vi "Diff_Drive_System_Act_AutoTune.vi"(6 "FPGA_Time_Seconds":dbl, 7 "Enabled":bool=TRUE, 9 "Right Speed":dbl, 10 "Left Speed":dbl, 11 "Diff_Drive_Device_Refs":T1 {"GyroDevRef"."Sample Rate" min=0.25 max=100.0 step=0.25}) -> ()   [LabVIEW 2019]
uses:
  <vilib>/Rock Robotics/WPI/ThirdParty/JAS_Junk/TrajLib/Trajectory_Library.lvlib
  Diff_Drive_System_Globals.vi
  <vilib>/Rock Robotics/SystemInterfaces/DIO/FPGA_DIOPWMChannel.ctl
  <vilib>/Rock Robotics/WPI/PWM/WPI_PWMDeadband.ctl
  <vilib>/Rock Robotics/WPI/MotorControl/WPI_MotorControlType.ctl
  <vilib>/Rock Robotics/SystemInterfaces/DIO/FPGA_DIOChannel.ctl
  <vilib>/Rock Robotics/WPI/MotorControl/WPI_MotorControlDeviceRef.ctl
  <vilib>/Rock Robotics/WPI/RobotDrive/WPI_RobotDriveDevRef.ctl
  <vilib>/Rock Robotics/SystemInterfaces/Encoder/FPGA_EncoderIdx.ctl
  <vilib>/Rock Robotics/WPI/Encoder/WPI_EncoderType.ctl
  <vilib>/Rock Robotics/SystemInterfaces/Counter/FPGA_CounterCtrSystemIndex.ctl
  <vilib>/Rock Robotics/WPI/Encoder/WPI_EncoderDevRef.ctl
  <vilib>/Rock Robotics/SystemInterfaces/spilib/spi_bus.ctl
  <vilib>/Rock Robotics/SystemInterfaces/AI/FPGA_AIChannel.ctl
  <vilib>/Rock Robotics/WPI/Gyro/WPI_GyroDevRef.ctl
  Diff_Drive_System_Device_Refs.ctl
panel:
  # "Analog"
  # "XRS"
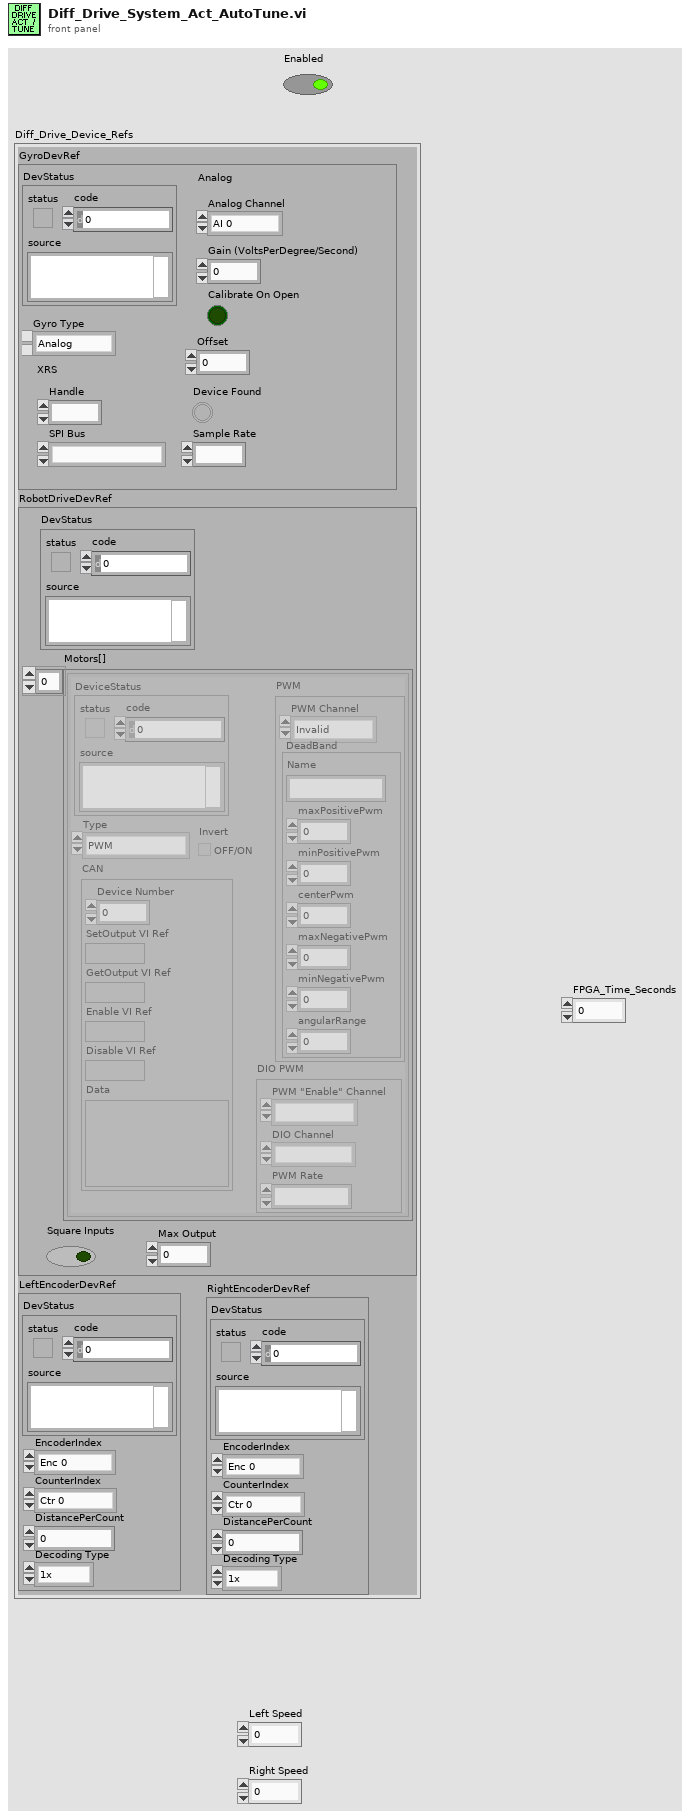
[diagram p1: front panel]
types:
  T1 = typedef "Diff_Drive_System_Device_Refs.ctl" = cluster{"GyroDevRef":T2, "RobotDriveDevRef":T5, "LeftEncoderDevRef":T11, "RightEncoderDevRef":T11}
  T2 = typedef "WPI_GyroDevRef.ctl" = cluster{"DevStatus":errorcluster, "Analog Channel":T3, "Gain (VoltsPerDegree/Second)":dbl, "Gyro Type":enum16{"Analog", "XRS450"}, "Handle":i32, "SPI Bus":T4, "Device Found":bool, "Sample Rate":dbl, "Calibrate On Open":bool, "Offset":dbl}
  T3 = typedef "FPGA_AIChannel.ctl" = enum8{"AI 0", "AI 1", "AI 2", "AI 3", "AI MXP 0", "AI MXP 1", "AI MXP 2", "AI MXP 3", "Invalid"}
  T4 = typedef "spi_bus.ctl" = enum16{"SPI On-Board, CS0", "SPI On-Board, CS1", "SPI On-Board, CS2", "SPI On-Board, CS3", "SPI MXP", "Invalid"}
  T5 = typedef "WPI_RobotDriveDevRef.ctl" = cluster{"DevStatus":errorcluster, "Motors[]":T6[], "Square Inputs":bool, "Max Output":dbl}
  T6 = typedef "WPI_MotorControlDeviceRef.ctl" = cluster{"DeviceStatus":errorcluster, "Type":T7, "PWM":cluster{"PWM Channel":T8, "DeadBand":T9}, "CAN":cluster{"Device Number":u8, "SetOutput VI Ref":variant, "GetOutput VI Ref":variant, "Enable VI Ref":variant, "Disable VI Ref":variant, "Data":variant}, "Invert":bool, "DIO PWM":cluster{"PWM \"Enable\" Channel":T8, "DIOChannel":T10, "PWM Rate":dbl}}
  T7 = typedef "WPI_MotorControlType.ctl" = enum16{"PWM", "CAN", "DIO PWM"}
  T8 = typedef "FPGA_DIOPWMChannel.ctl" = enum8{"PWM 0", "PWM 1", "PWM 2", "PWM 3", "PWM 4", "PWM 5", "PWM 6", "PWM 7", "PWM 8", "PWM 9", "PWM MXP 0", "PWM MXP 1", "PWM MXP 2", "PWM MXP 3", "PWM MXP 4", "PWM MXP 5", "PWM MXP 6", "PWM MXP 7", "PWM MXP 8", "PWM MXP 9", "Invalid"}
  T9 = typedef "WPI_PWMDeadband.ctl" = cluster{"Name":string, "maxPositivePwm":i32, "minPositivePwm":i32, "centerPwm":i32, "maxNegativePwm":i32, "minNegativePwm":i32, "angularRange":u16}
  T10 = typedef "FPGA_DIOChannel.ctl" = enum8{"DIO 0", "DIO 1", "DIO 2", "DIO 3", "DIO 4", "DIO 5", "DIO 6", "DIO 7", "DIO 8", "DIO 9", "DIO MXP 0", "DIO MXP 1", "DIO MXP 2", "DIO MXP 3", "DIO MXP 4", "DIO MXP 5", "DIO MXP 6", "DIO MXP 7", "DIO MXP 8", "DIO MXP 9", "DIO MXP 10", "DIO MXP 11", "DIO MXP 12", "DIO MXP 13", "DIO MXP 14", "DIO MXP 15", "SPI Port CS1", "SPI Port CS2", "SPI Port CS3", "SPI Port MISO", "SPI Port MOSI", "Invalid"}
  T11 = typedef "WPI_EncoderDevRef.ctl" = cluster{"DevStatus":errorcluster, "EncoderIndex":T12, "CounterIndex":T13, "DistancePerCount":dbl, "Decoding Type":T14}
  T12 = typedef "FPGA_EncoderIdx.ctl" = enum8{"Enc 0", "Enc 1", "Enc 2", "Enc 3", "Enc 4", "Enc 5", "Enc 6", "Enc 7", "Invalid"}
  T13 = typedef "FPGA_CounterCtrSystemIndex.ctl" = enum8{"Ctr 0", "Ctr 1", "Ctr 2", "Ctr 3", "Ctr 4", "Ctr 5", "Ctr 6", "Ctr 7", "Invalid"}
  T14 = typedef "WPI_EncoderType.ctl" = enum16{"1x", "2x", "4x"}
  T15 = enum16{"Ziegler Nicols - Fast", "Ziegler Nicols - Normal", "Ziegler Nicols - Slow", "CHR regulator - 0% overshoot", "CHR regulator - 20% overshoot", "CHR servo - 0 % overshoot", "CHR servo - 20% overshoot"}
  T16 = typedef "Trajectory_Library.lvlib/SIMPLE_MOTOR_FF.ctl" = cluster{"Ks":dbl, "Kv":dbl, "Ka":dbl, "KnInv":dbl}
  T17 = typedef "Trajectory_Library.lvlib/PID_ADV_LIMITS.ctl" = cluster{"MaxInput":dbl, "MinInput":dbl, "Continuous":bool, "MaxOutput":dbl, "MinOutput":dbl}
  T18 = typedef "Trajectory_Library.lvlib/PID_ADV_TUNING.ctl" = cluster{"Kf":dbl, "Kp":dbl, "Ki":dbl, "Kd":dbl, "MaximumIntegral":dbl, "MinimumIntegral":dbl, "Filter Derivative":bool}
  T19 = cluster{"Controller Constant Type":enum16{"Ziegler Nicols - Fast", "Ziegler Nicols - Normal", "Ziegler Nicols - Slow", "CHR regulator - 0% overshoot", "CHR regulator - 20% overshoot", "CHR servo - 0 % overshoot", "CHR servo - 20% overshoot"}, "Type of Controller":enum16{"P", "PI", "PID"}, "CO Offset":dbl, "Kn":dbl, "Tuning Tolerance":dbl, "Plant Tolerance":dbl, "Newest Avg Time ":i32, "Long Ave Time":i32}
  T20 = cluster{"proportional gain (Kp)":dbl, "integral time (Ki / Sec)":dbl, "derivative time (Kd /Sec)":dbl}
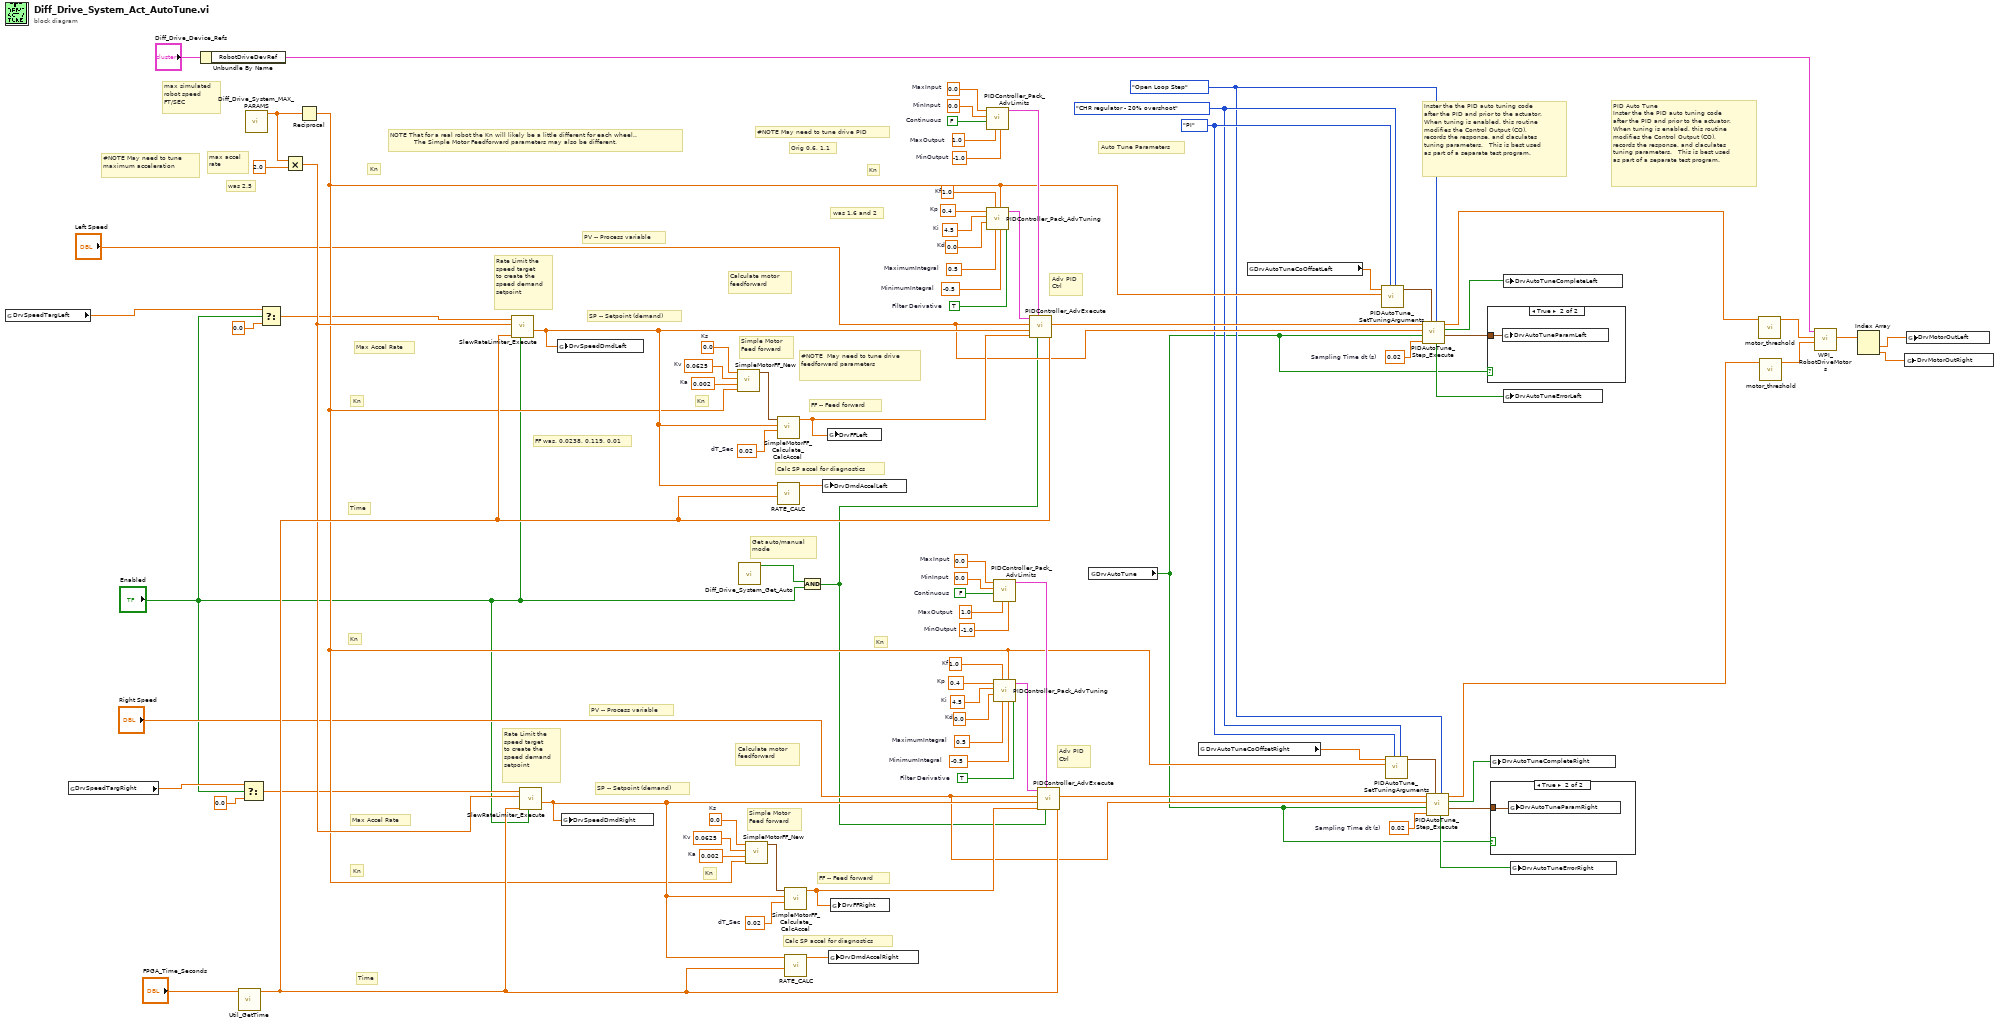
[diagram p0: block diagram]
diagram:
  w28 = 0.02  # Sampling Time dt (s)
  w13 = enum16{"Open Loop Step", "Closed Loop Step"}."Open Loop Step" ("Procedure Type")
  w14 = T15."CHR regulator - 20% overshoot" ("Controller Constant Type")
  w15 = enum16{"P", "PI", "PID"}."PI" ("Type of Controller")
  w33 = 0.02  # Sampling Time dt (s)
  w52 = 0.4  # Kp
  w51 = 4.5  # Ki
  w50 = 0.0  # Kd
  w49 = 1.0  # Kf
  w48 = 0.5  # MaximumIntegral
  w47 = -0.5  # MinimumIntegral
  w46 = TRUE  # Filter Derivative
  w44 = 0.0  # MinInput
  w43 = FALSE  # Continuous
  w42 = 1.0  # MaxOutput
  w45 = -1.0  # MinOutput
  w41 = 0.0  # MaxInput
  w57 = 0.02  # dT_Sec
  w55 = 0.0  # Ks
  w54 = 0.0625  # Kv
  w53 = 0.002  # Ka
  w75 = 0.4  # Kp
  w74 = 4.5  # Ki
  w73 = 0.0  # Kd
  w72 = 1.0  # Kf
  w71 = 0.5  # MaximumIntegral
  w70 = -0.5  # MinimumIntegral
  w69 = TRUE  # Filter Derivative
  w67 = 0.0  # MinInput
  w66 = FALSE  # Continuous
  w65 = 1.0  # MaxOutput
  w68 = -1.0  # MinOutput
  w64 = 0.0  # MaxInput
  w80 = 0.02  # dT_Sec
  w78 = 0.0  # Ks
  w77 = 0.0625  # Kv
  w76 = 0.002  # Ka
  # "PID Auto Tune\nInster the the PID auto tuning code\nafter the PID and prior to the actuator.\nWhen tuning is enabled, this routine\nmodifies the Control Output (CO), \nrecords the response, and claculates\ntuning parameters.   This is best used\nas part of a separate test program."
  # "was 1.6 and 2"
  # "Auto Tune Parameters"
  # "Inster the the PID auto tuning code\nafter the PID and prior to the actuator.\nWhen tuning is enabled, this routine\nmodifies the Control Output (CO), \nrecords the response, and claculates\ntuning parameters.   This is best used\nas part of a separate test program."
  # "Get auto/manual\nmode"
  # "FF was, 0.0238, 0.119, 0.01"
  # "Orig 0.6, 1.1"
  # "NOTE That for a real robot the Kn will likely be a little different for each wheel..\n            The Simple Motor Feedforward parameters may also be different."
  # "Max Accel Rate"
  # "Max Accel Rate"
  # "Time"
  # "Kn"
  # "Kn"
  # "Kn"
  # "Kn"
  # "Time"
  # "Kn"
  # "PV -- Process variable"
  # "Kn"
  # "Calc SP accel for diagnostics"
  # "FF -- Feed forward"
  # "SP -- Setpoint (demand)"
  # "Adv PID\nCtrl"
  # "Calculate motor\nfeedforward"
  # "Rate Limit the \nspeed target\nto create the\nspeed demand\nsetpoint"
  # "Simple Motor\nFeed forward"
  # "Kn"
  # "PV -- Process variable"
  # "Kn"
  # "Calc SP accel for diagnostics"
  # "FF -- Feed forward"
  # "SP -- Setpoint (demand)"
  # "Adv PID\nCtrl"
  # "Calculate motor\nfeedforward"
  # "was 2.5"
  # "Rate Limit the \nspeed target\nto create the\nspeed demand\nsetpoint"
  # "Simple Motor\nFeed forward"
  # "#NOTE May need to tune drive PID"
  # "#NOTE May need to tune maximum acceleration"
  # "#NOTE  May need to tune drive feedforward parameters"
  # "max simulated\nrobot speed\nFT/SEC"
  # "max accel\nrate"
  n1 = global read "Diff_Drive_System_Globals.vi" "DrvSpeedTargLeft"() -> (w4:dbl)
  n2 = global read "Diff_Drive_System_Globals.vi" "DrvSpeedTargRight"() -> (w6:dbl)
  n3 = Unbundle By Name("Diff_Drive_Device_Refs") -> ("RobotDriveDevRef"=w83:T5)
  n4 = call <vilib>:"Util_GetTime.vi"("Pass_Through_Time"="FPGA_Time_Seconds") -> ("FPGA_Time_Seconds"=w38:dbl)  [unwired: 8 in, 2 out]
  n5 = Select(t=w6, s="Enabled", f=0.0) -> (s? t:f=w7:dbl)
  n6 = call "Diff_Drive_System_MAX_PARAMS.vi"() -> ("Max Speed Ft/Sec"=w59:dbl)  [unwired: 9 in, 2 out]
  n7 = Select(t=w4, s="Enabled", f=0.0) -> (s? t:f=w3:dbl)
  n8 = Multiply(x=w59, y=2.0 ("x")) -> (x*y=w37:dbl)
  n9 = Reciprocal(x=w59) -> (1/x=w23:dbl)
  n10 = call <vilib>:"SlewRateLimiter_Execute.vi"("Enable"="Enabled", "Time"=w38, "PositiveRate"=w37, "Input"=w3) -> ("Output"=w61:dbl)  [unwired: 6 in, 1 out]
  n11 = call <vilib>:"SlewRateLimiter_Execute.vi"("Enable"="Enabled", "Time"=w38, "PositiveRate"=w37, "Input"=w7) -> ("Output"=w34:dbl)  [unwired: 6 in, 1 out]
  n12 = global write "Diff_Drive_System_Globals.vi" "DrvSpeedDmdLeft"(w61) -> ()
  n13 = global write "Diff_Drive_System_Globals.vi" "DrvSpeedDmdRight"(w34) -> ()
  n14 = call <vilib>:"SimpleMotorFF_New.vi"("Kn"=w23, "Ka"=w76, "Kv"=w77, "Ks"=w78) -> ("SIMPLE_MOTOR_FF"=w79:T16)  [unwired: 7 in]
  n15 = call "Diff_Drive_System_Get_Auto.vi"() -> ("Auto Mode"=w10:bool)  [unwired: 11 in]
  n16 = call <vilib>:"SimpleMotorFF_New.vi"("Kn"=w23, "Ka"=w53, "Kv"=w54, "Ks"=w55) -> ("SIMPLE_MOTOR_FF"=w56:T16)  [unwired: 7 in]
  n17 = call <vilib>:"SimpleMotorFF_Calculate_CalcAccel.vi"("dT_Sec"=w80, "VelSp"=w61, "SIMPLE_MOTOR_FF"=w79) -> ("FeedForward"=w58:dbl)  [unwired: 8 in]
  n18 = call "RATE_CALC.vi"("Time"=w38, "Input"=w61) -> ("Output"=w60:dbl)  [unwired: 9 in]
  n19 = call <vilib>:"SimpleMotorFF_Calculate_CalcAccel.vi"("dT_Sec"=w57, "VelSp"=w34, "SIMPLE_MOTOR_FF"=w56) -> ("FeedForward"=w36:dbl)  [unwired: 8 in]
  n20 = call "RATE_CALC.vi"("Time"=w38, "Input"=w34) -> ("Output"=w35:dbl)  [unwired: 9 in]
  n21 = And(x=w10, y="Enabled") -> (x .and. y?=w9:bool)
  n22 = global write "Diff_Drive_System_Globals.vi" "DrvDmdAccelLeft"(w60) -> ()
  n23 = global write "Diff_Drive_System_Globals.vi" "DrvFFLeft"(w58) -> ()
  n24 = global write "Diff_Drive_System_Globals.vi" "DrvDmdAccelRight"(w35) -> ()
  n25 = global write "Diff_Drive_System_Globals.vi" "DrvFFRight"(w36) -> ()
  n26 = call <vilib>:"PIDController_Pack_AdvLimits.vi"("MinOutput"=w68, "MaxOutput"=w65, "Continuous"=w66, "MinInput"=w67, "MaxInput"=w64) -> ("Adv PID Limits"=w62:T17)  [unwired: 6 in]
  n27 = call <vilib>:"PIDController_Pack_AdvTuning.vi"("Filter Derivative"=w69, "MinimumIntegral"=w70, "Kn"=w23, "MaximumIntegral"=w71, "Kf"=w72, "Kd"=w73, "Ki"=w74, "Kp"=w75) -> ("Adv PID Tuning"=w63:T18)  [unwired: 3 in]
  n28 = call <vilib>:"PIDController_Pack_AdvLimits.vi"("MinOutput"=w45, "MaxOutput"=w42, "Continuous"=w43, "MinInput"=w44, "MaxInput"=w41) -> ("Adv PID Limits"=w39:T17)  [unwired: 6 in]
  n29 = call <vilib>:"PIDController_Pack_AdvTuning.vi"("Filter Derivative"=w46, "MinimumIntegral"=w47, "Kn"=w23, "MaximumIntegral"=w48, "Kf"=w49, "Kd"=w50, "Ki"=w51, "Kp"=w52) -> ("Adv PID Tuning"=w40:T18)  [unwired: 3 in]
  n30 = call <vilib>:"PIDController_AdvExecute.vi"("Time"=w38, "Auto"=w9, "Adv PID Limits"=w62, "FF-FeedForward"=w58, "SP-SetPoint"=w61, "PV-Measurement"="Left Speed", "Adv PID Tuning"=w63) -> ("CO-ControlOutput"=w30:dbl)  [unwired: 2 in, 2 out]
  n31 = call <vilib>:"PIDController_AdvExecute.vi"("Time"=w38, "Auto"=w9, "Adv PID Limits"=w39, "FF-FeedForward"=w36, "SP-SetPoint"=w34, "PV-Measurement"="Right Speed", "Adv PID Tuning"=w40) -> ("CO-ControlOutput"=w26:dbl)  [unwired: 2 in, 2 out]
  n32 = global read "Diff_Drive_System_Globals.vi" "DrvAutoTune"() -> (w11:bool)
  n33 = global read "Diff_Drive_System_Globals.vi" "DrvAutoTuneCoOffsetRight"() -> (w24:dbl)
  n34 = global read "Diff_Drive_System_Globals.vi" "DrvAutoTuneCoOffsetLeft"() -> (w1:dbl)
  n35 = call <vilib>:"PIDAutoTune_SetTuningArguments.vi"("Controller Constant Type"=w14, "Type of Controller"=w15, "Kn"=w23, "CO Offset"=w1) -> ("Configuration Parameters"=w32:T19)  [unwired: 7 in]
  n36 = call <vilib>:"PIDAutoTune_SetTuningArguments.vi"("Controller Constant Type"=w14, "Type of Controller"=w15, "Kn"=w23, "CO Offset"=w24) -> ("Configuration Parameters"=w27:T19)  [unwired: 7 in]
  n37 = call <vilib>:"PIDAutoTune_Step_Execute.vi"("Procedure Type"=w13, "Configuration Parameters"=w32, "Sampling Time dt (s)"=w33, "Tune"=w11, "Measurement  (PV)"="Left Speed", "Control Output (Co)"=w30) -> ("New Tuning Parameters"=w21:T20, "Tuning Done"=w22:bool, "Adj CO"=w29:dbl, "Error Occured"=w12:bool)  [unwired: 2 out]
  n38 = call <vilib>:"PIDAutoTune_Step_Execute.vi"("Procedure Type"=w13, "Configuration Parameters"=w27, "Sampling Time dt (s)"=w28, "Tune"=w11, "Measurement  (PV)"="Right Speed", "Control Output (Co)"=w26) -> ("New Tuning Parameters"=w19:T20, "Tuning Done"=w20:bool, "Adj CO"=w25:dbl, "Error Occured"=w16:bool)  [unwired: 2 out]
  n39 = case shown="True" w11 {
    tunnel: w21 -> [_ w89]
    frame False {
    }
    frame True {
      n40 = global write "Diff_Drive_System_Globals.vi" "DrvAutoTuneParamLeft"(w89) -> ()
    }
  }
  n41 = global write "Diff_Drive_System_Globals.vi" "DrvAutoTuneCompleteRight"(w20) -> ()
  n42 = case shown="True" w11 {
    tunnel: w19 -> [_ w90]
    frame False {
    }
    frame True {
      n43 = global write "Diff_Drive_System_Globals.vi" "DrvAutoTuneParamRight"(w90) -> ()
    }
  }
  n44 = global write "Diff_Drive_System_Globals.vi" "DrvAutoTuneCompleteLeft"(w22) -> ()
  n45 = global write "Diff_Drive_System_Globals.vi" "DrvAutoTuneErrorLeft"(w12) -> ()
  n46 = global write "Diff_Drive_System_Globals.vi" "DrvAutoTuneErrorRight"(w16) -> ()
  n47 = call "motor_threshold.vi"("motor in"=w29) -> ("motor out"=w31:dbl)  [unwired: 10 in]
  n48 = call "motor_threshold.vi"("motor in"=w25) -> ("motor out"=w87:dbl)  [unwired: 10 in]
  n49 = call <vilib>:"WPI_RobotDriveMotors.vi"("RightSpeed"=w87, "LeftSpeed"=w31, "RobotDriveDevRef"=w83) -> ("Motor Values"=w86:dbl[])  [unwired: 6 in, 2 out]
  n50 = Index Array(array=w86) -> (element #1=w82:dbl, element #2=w81:dbl)  [unwired: 2 in]
  n51 = global write "Diff_Drive_System_Globals.vi" "DrvMotorOutRight"(w81) -> ()
  n52 = global write "Diff_Drive_System_Globals.vi" "DrvMotorOutLeft"(w82) -> ()
